vi "Check and Override Channel Configuration.vi"(8 "error in (no error)":errorcluster, 10 "Custom Config Data in":u8[](array[numeric]) format="%.0x", 11 "CIFFIFO in":refnum<class "CIF_Iceoryx_PCAP_Universal.lvclass">) -> (0 "error out":errorcluster, 2 "Custom Config Data out":u8[](array[numeric]) format="%.0x", 3 "CIFFIFO out":refnum<class "CIF_Iceoryx_PCAP_Universal.lvclass">)   [LabVIEW 2021, in "CIF_Iceoryx_PCAP_Universal.lvclass"]
uses:
  CIF_Iceoryx_PCAP_Universal.lvclass
  ChannelCommon/ChannelCommon.lvlib
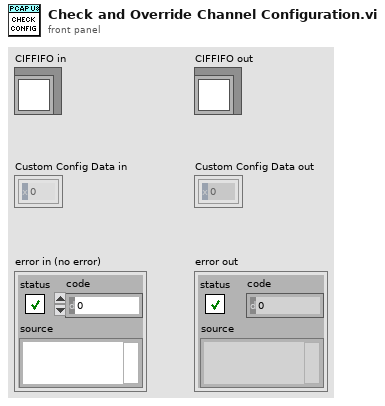
[diagram p1: front panel]
types:
  T1 = typedef "ChannelCommon.lvlib/FIFO Config Extended.ctl" = cluster{"Max Bytes/Msg":u64, "Max Msg/FIFO":u64, "Flags":u64, "Best Effort Subscribers":u32, "Backpressure Subscribers":u32, "Custom Data":u8[]}
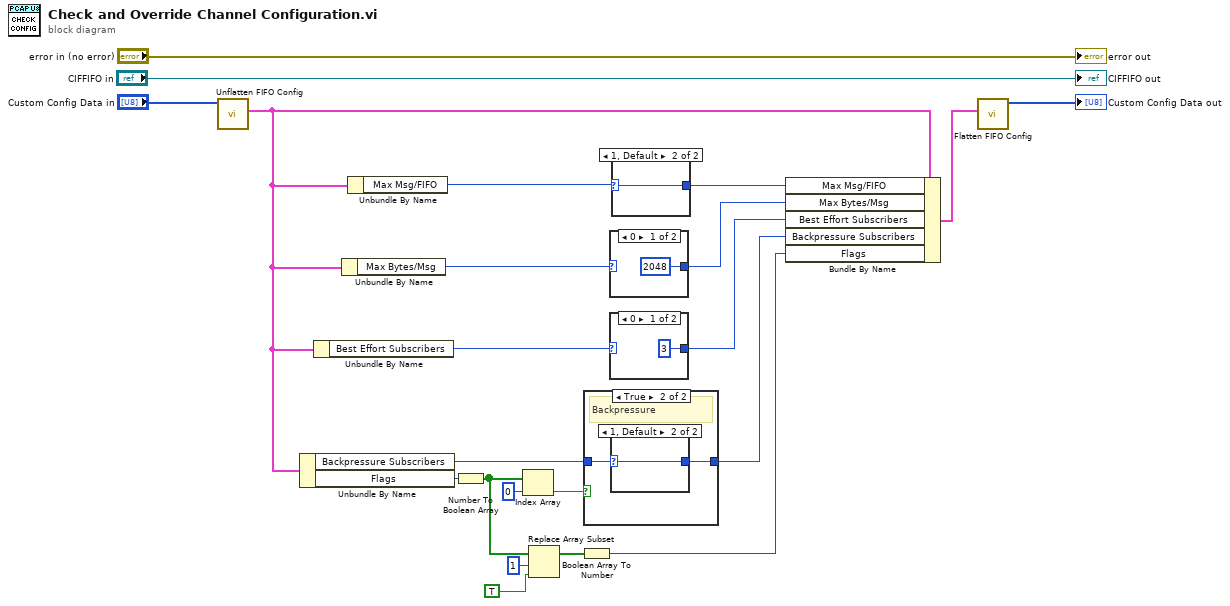
[diagram p0: block diagram]
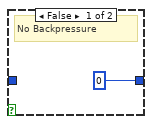
[diagram p2: hidden frame]
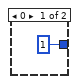
[diagram p3: hidden frame]
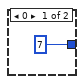
[diagram p6: hidden frame]
diagram:
  n1 = call "Unflatten FIFO Config.vi"("Flattened Data in"="Custom Config Data in") -> ("FIFO Config Extended in"=w12:T1)  [unwired: 8 in, 2 out]
  n2 = Unbundle By Name(w12) -> ("Backpressure Subscribers"=w7:u32, "Flags"=w13:u64)
  n3 = Unbundle By Name(w12) -> ("Best Effort Subscribers"=w11:u32)
  n4 = Unbundle By Name(w12) -> ("Max Bytes/Msg"=w19:u64)
  n5 = Unbundle By Name(w12) -> ("Max Msg/FIFO"=w18:u64)
  n6 = Number To Boolean Array(number=w13) -> (Boolean array=w5:bool[])
  n7 = Index Array(array=w5, index=0) -> (element=w8:bool)
  n8 = Replace Array Subset(array=w5, new element=TRUE ("new element/subarray"), index=1) -> (w2:bool[])
  n9 = Boolean Array To Number(Boolean array=w2) -> (number=w1:u64)
  n10 = case shown="True" w8 {
    tunnel: w7 -> [_ w25]
    tunnel: [u32 0 ("Best Effort Subscribers") w24] -> w6
    frame False {
      # "No Backpressure"
    }
    frame True {
      # "Backpressure"
      n11 = case shown="1, Default" w25 {
        selector: w25 -> [_ w27]
        tunnel: [u32 1 ("y") w27] -> w24
        frame 0 {
        }
        frame 1, Default {
        }
      }
    }
  }
  n12 = case shown="0" w19 {
    selector: w19 -> [_ w29]
    tunnel: [u64 2048 ("y") w29] -> w16
    frame 0 {
    }
    frame 1, Default {
    }
  }
  n13 = case shown="0" w11 {
    selector: w11 -> [_ w31]
    tunnel: [u32 3 ("y") w31] -> w10
    frame 0 {
    }
    frame 1, Default {
    }
  }
  n14 = case shown="1, Default" w18 {
    selector: w18 -> [_ w33]
    tunnel: [u64 7 ("y") w33] -> w17
    frame 0 {
    }
    frame 1, Default {
    }
  }
  n15 = Bundle By Name(cluster=w12, "Max Msg/FIFO"=w17, "Max Bytes/Msg"=w16, "Best Effort Subscribers"=w10, "Backpressure Subscribers"=w6, "Flags"=w1) -> (w14:T1)
  n16 = call "Flatten FIFO Config.vi"("FIFO Config Extended in"=w14) -> ("Flattened FIFO Config"=→"Custom Config Data out":u8[])  [unwired: 10 in]
  "error out" <- "error in (no error)"
  "CIFFIFO out" <- "CIFFIFO in"
